vi "DialogManageInterfaces.vi"(8 "error in (no error)":errorcluster, 10 "ClassItemRefIn":refnum<vi>, 11 "ClassWriterNativeIn":refnum<class "ClassWriterNative.lvclass">) -> (0 "error out":errorcluster, 1 "HanldeInterfacesData":T1, 2 "Cancelled":bool, 3 "ClassWriterNativeOut":refnum<class "ClassWriterNative.lvclass">)   [LabVIEW 2020, in "ClassWriterNative.lvclass"]
uses:
  <resource>/Framework/Providers/Open_GDS/ClassProviders/Provider_LvNativeClass/ClassWriterNative_class/ClassWriterNative.lvclass
  <resource>/Framework/Providers/Open_GDS/ClassProviders/Provider_BaseClassInterface/ClassWriter_class/HandleInterfacesData.ctl
  <resource>/Framework/Providers/Open_GDS/ClassProviders/Common/InterfaceLibrary/InterfaceInfo.ctl
  <resource>/Framework/Providers/Open_GDS/ClassProviders/Common/LvClass_class/GDSLvClass_ClassMethodInfo.ctl
  <resource>/Framework/Providers/Open_GDS/ClassProviders/Provider_BaseClassInterface/ClassWriter_class/InterfacesToImplement.ctl
  <resource>/Framework/Providers/Open_GDS/ClassProviders/Common/LvClass_class/GDSLvClass_ClassInfo.ctl
  <vilib>/picture/picture.llb/imagedata.ctl
  <vilib>/Utility/miscctls.llb/LVRowAndColumnTypeDef.ctl
  <vilib>/Utility/miscctls.llb/LVRowAndColumnUnsignedTypeDef.ctl
  faae8295-b5d0-4054-ba26-443edd8c351b.vi
  a5869a5e-804e-44c9-8055-a166d2e26855.vi
  516f7541-512c-4146-8a63-54cd49fe1b68.vi
  c799aba2-3e95-4f13-9023-21e7452f1ffd.vi
  <resource>/Framework/Providers/Open_GDS/ClassProviders/Provider_LvNativeClass/ClassWriterNative_class/ClassWriterNative.lvclass/ClassWriterNative.ctl
  <resource>/Framework/Providers/Open_GDS/ClassProviders/Common/InterfaceLibrary/InterfaceLibrary.lvlib
  <resource>/Framework/Providers/Open_GDS/ClassProviders/Provider_BaseClassInterface/ClassWriter_class/ClassWriter.lvclass
  <resource>/Framework/Providers/_ClassSupport/Class Provider Support.lvlib
panel:
  in  "Tree":string(tree) caption="No methods selected"
  in  "_ShowContextHelp":bool
  in  "Help":bool
  in  "Cancel":bool
  in  "Save":bool
  out "ProductPicture":picture
  out "InterfaceList":i32[](listbox)
  in  "InterfaceFilter":string caption="Filter"
  out "Class":string
  # "Select Parent Interfaces (tick or untick check box)"
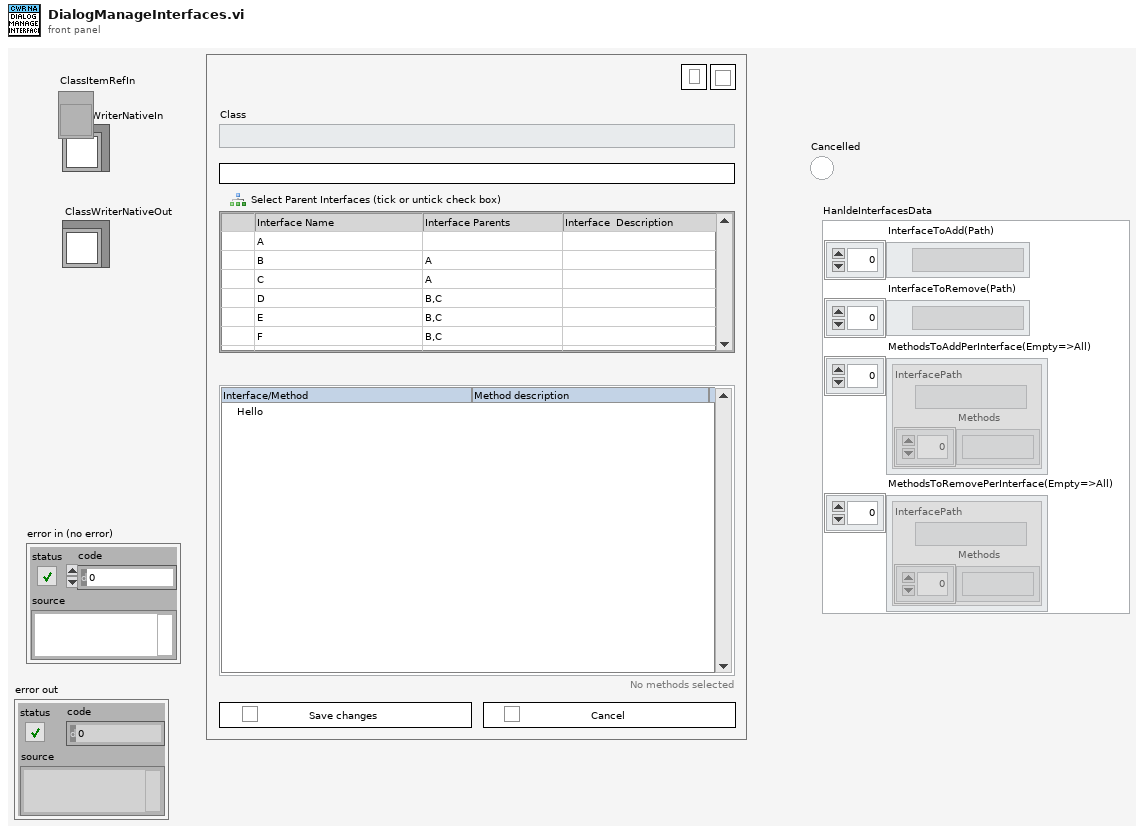
[diagram p1: front panel]
types:
  T1 = typedef "ClassWriter.lvclass/HandleInterfacesData.ctl" = cluster{"InterfaceToAdd(Path)":path[], "InterfaceToRemove(Path)":path[], "MethodsToAddPerInterface(Empty=>All)":cluster{"InterfacePath":path, "Methods":string[]}[], "MethodsToRemovePerInterface(Empty=>All)":cluster{"InterfacePath":path, "Methods":string[]}[]}
  T2 = cluster{"Font Name":string, "Size":u16, "Bold":bool, "Italic":bool, "Underline":bool, "Strikeout":bool, "Color":u32}
  T3 = typedef "InterfaceLibrary.lvlib/InterfaceInfo.ctl" = cluster{"Name(Short if no Conflicts)":string, "FullQualifierName":string, "Description":string, "Path":path, "ParentInterfaceNames(Short if no Conflitcs)":string[], "ParentInterfaceFullQualifierNames":string[], "IconPath":path, "Methods":T4[], "DynamicDispatchMethod":bool[]}
  T4 = typedef "GDSLvClass_ClassMethodInfo.ctl" = cluster{"Name":string, "Descriptions":string, "RelativePath":path, "SourceScope":enum32{"invalid scope", "public", "private", "protected", "community"}, "MustOverride":bool, "VirtualFolderLocation":string[], "DynamicDispatch":bool}
  T5 = typedef "ClassWriter.lvclass/InterfacesToImplement.ctl" = cluster{"InterfacePath":path[], "CreateMethods":bool, "MethodsPerInterface(Empty=>All)":cluster{"Methods":string[]}[]}
  T6 = typedef "GDSLvClass_ClassInfo.ctl" = cluster{"Path":path, "Name":string, "QualifiedName":string}
  T7 = cluster{"Cancel":bool, "InterfaceInfo":T3[], "IsInterface?":bool, "ParentInterfaces(path)":path[], "Interfaces(MethodsImplemented)":cluster{"Methods":string[]}[], "InterfaceIcons":path[], "VisiableInterfaceIndexes":i32[], "InterfaceSelection":enum16{"Empty", "Not", "Grey", "Blue"}[], "DisabledInterfaceIndexes":i32[], "InterfaceToAdd":T5, "InterfaceToRemove":T5, "MethodsSelectedPerInt":cluster{"Array":bool[]}[], "MethodsPerInterfaces":cluster{"Array":string[]}[], "Interfaces":string[], "StartInterfaceSelection":bool[], "Path":path, "DisabledInterafaces":i32[], "MethodsDisabledPerInt":cluster{"Array":bool[]}[], "SelectedInterfaceIndex":i32[], "ClassInheritanceHierarchy":T6[], "InterfacesParentClasesUses(path)":path[], "LvClasses":refnum<vi>[], "LvInterfaces":refnum<vi>[], "HandleInterfacesData":T1}
  T8 = typedef "imagedata.ctl" = cluster{"image type":i32, "image depth":i32, "image":u8[], "mask":u8[], "colors":u32[], "Rectangle":cluster{"left":i16, "top":i16, "right":i16, "bottom":i16}}
  T9 = typedef "LVRowAndColumnTypeDef.ctl" = cluster{"Row":i32, "Column":i32}
  T10 = typedef "LVRowAndColumnUnsignedTypeDef.ctl" = cluster{"Row":u32, "Column":u32}
  T11 = cluster{"FullQualifierInterfaceName":string, "MethodNames":string[]}[]
  T12 = cluster{"InterfacePath":path, "Methods":string[]}
  T13 = cluster{"ParentInterfaceFullQualifierNames":string[]}
  T14 = cluster{"FullQualifierName":string, "Methods":string[]}
  T15 = typedef "LVPoint32TypeDef.ctl" = cluster{"Horizontal":i32, "Vertical":i32}
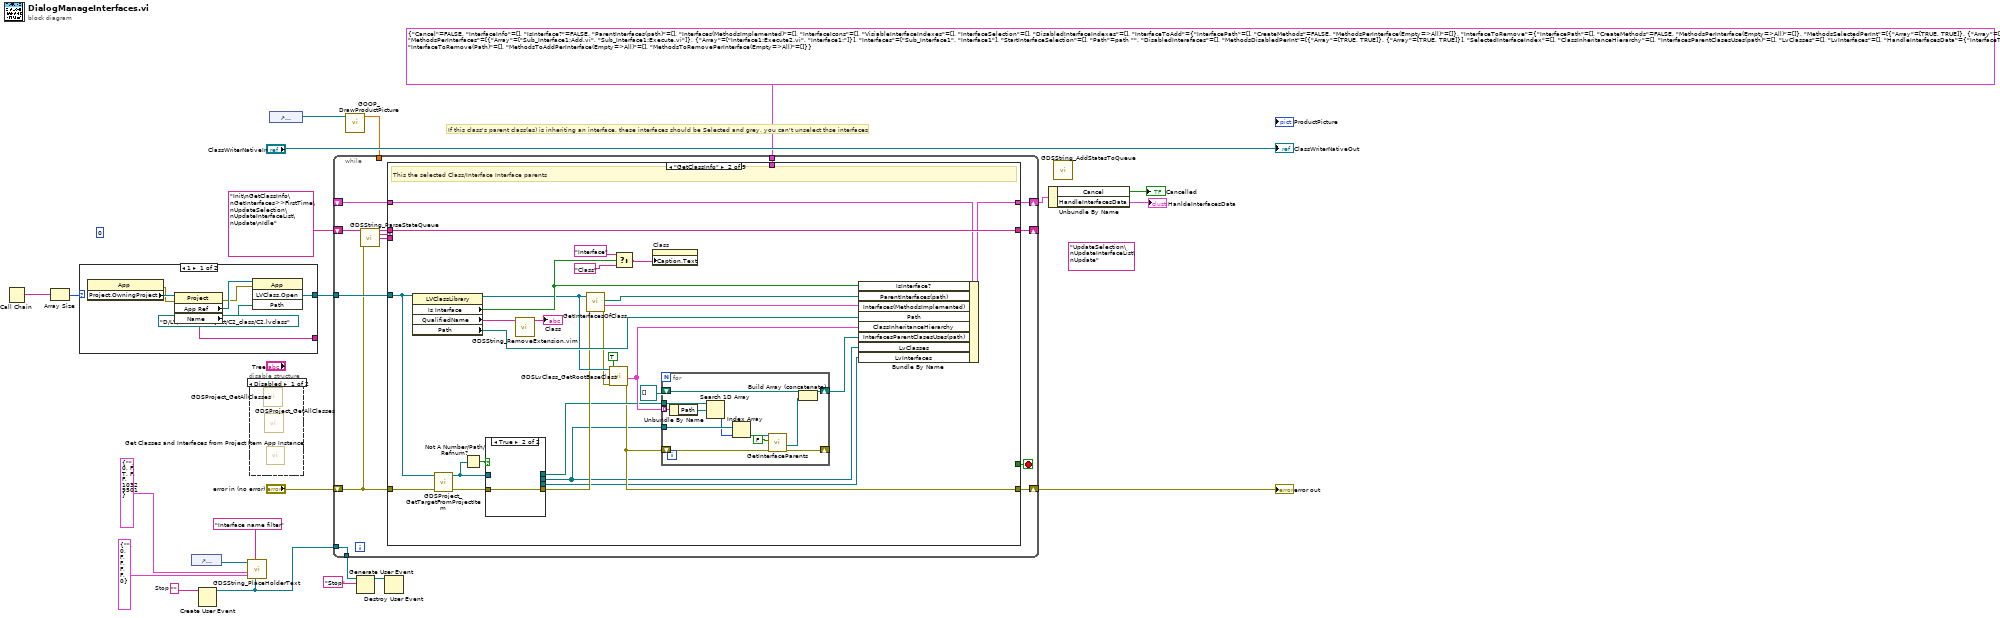
[diagram p0: block diagram]
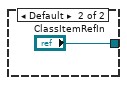
[diagram p3: hidden frame]
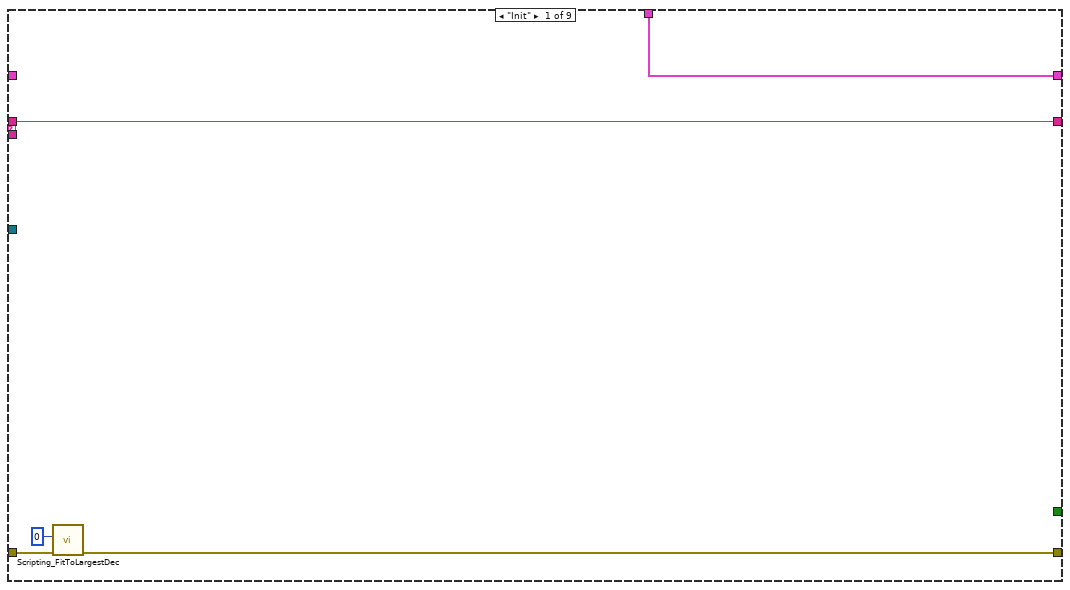
[diagram p4: hidden frame]
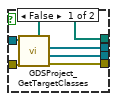
[diagram p5: hidden frame]
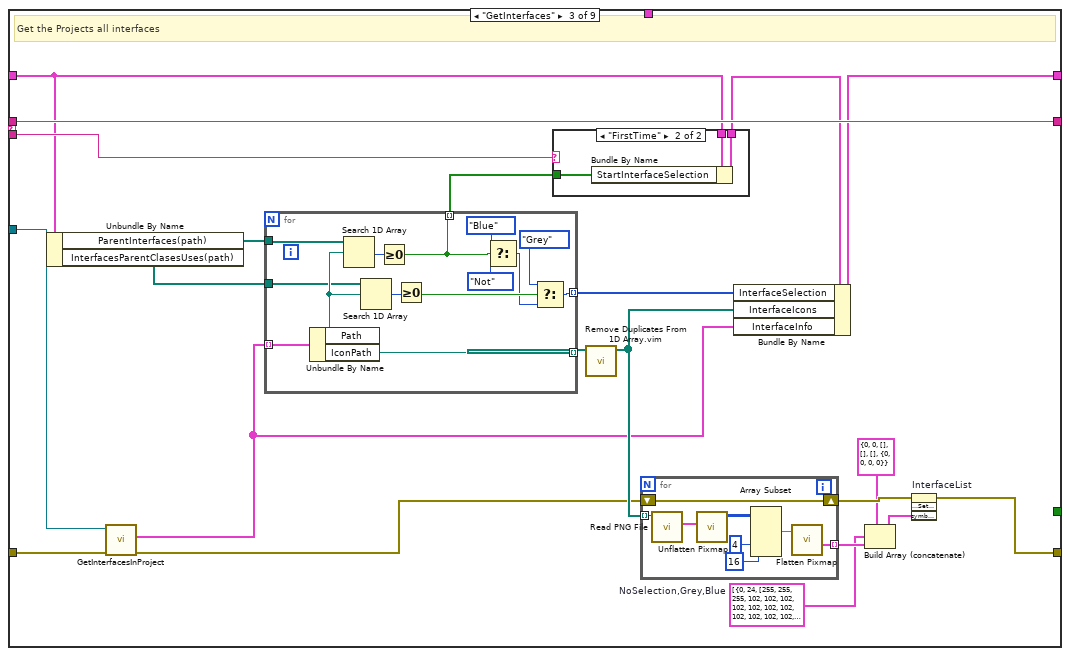
[diagram p6: hidden frame]
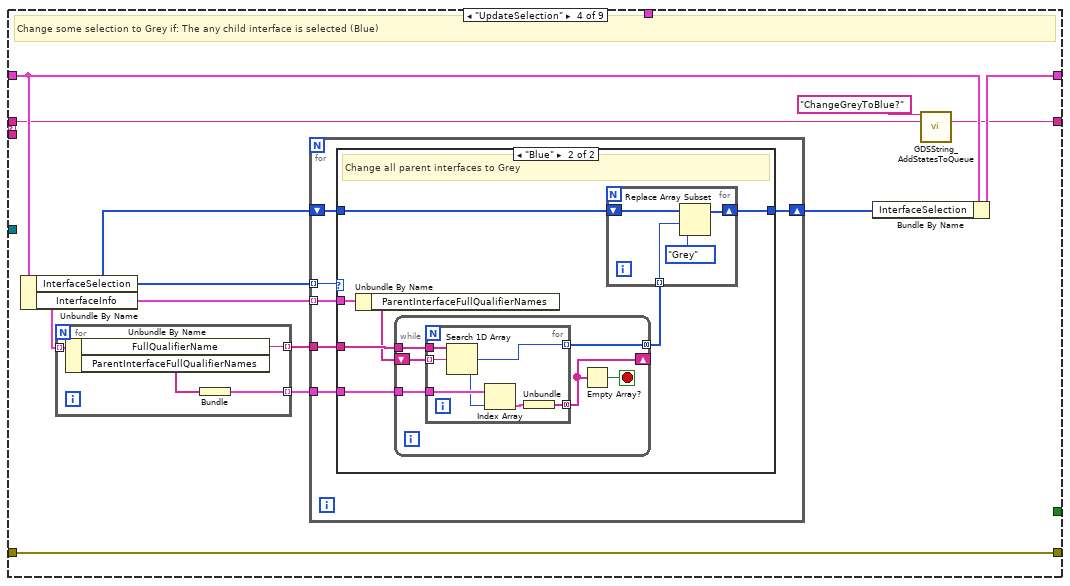
[diagram p8: hidden frame]
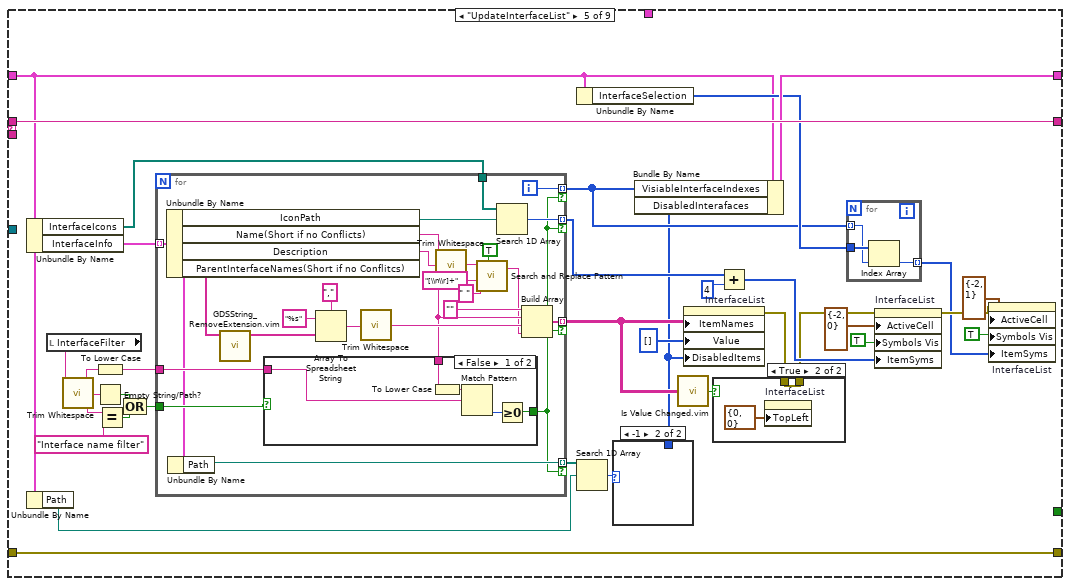
[diagram p10: hidden frame]
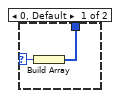
[diagram p11: hidden frame]
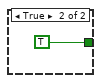
[diagram p13: hidden frame]
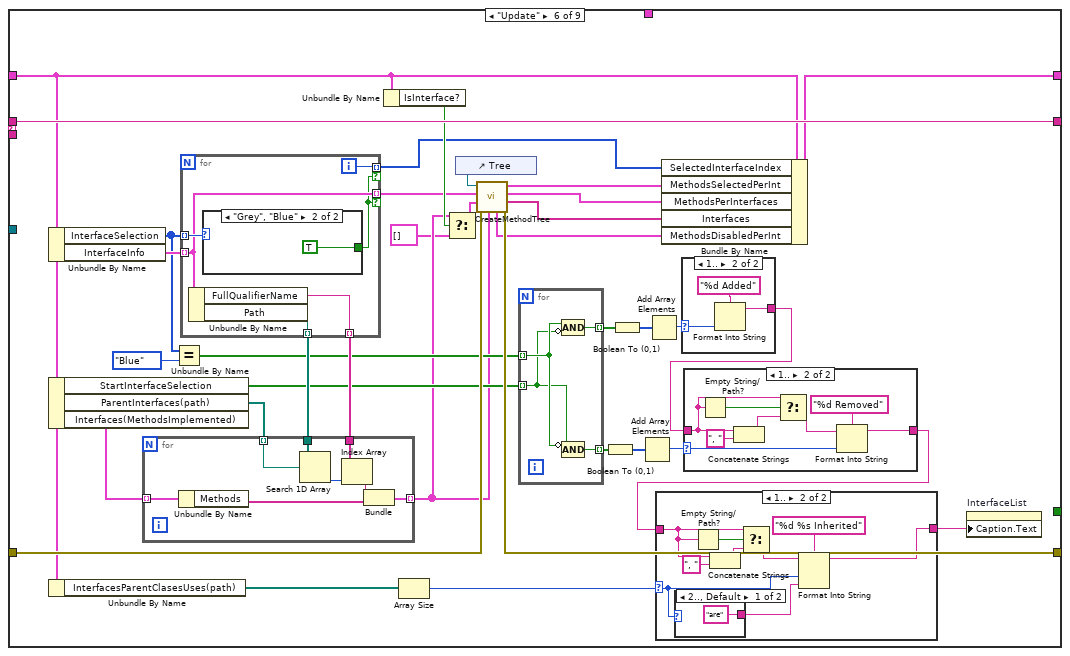
[diagram p14: hidden frame]
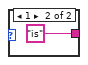
[diagram p16: hidden frame]
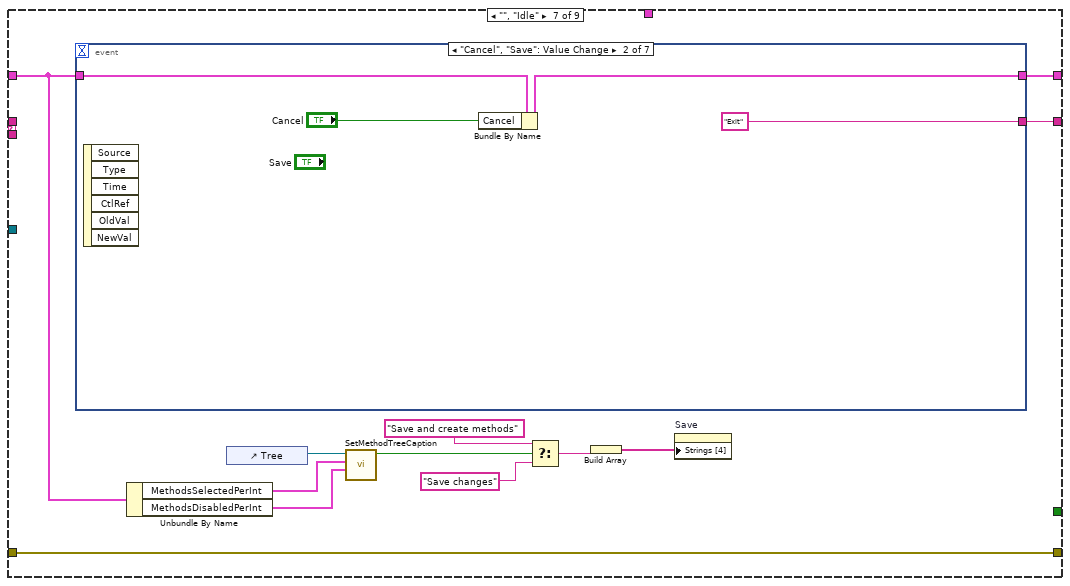
[diagram p20: hidden frame]
diagram:
  (unwired) 0
  w6 = ""  # Stop
  (unwired) "UpdateSelection\nUpdateInterfaceList\nUpdate"
  # "If this class's parent class(es) is inheriting an interface, these interfaces should be Selected and grey, you can't unselect thse interfaces"
  n1 = Call Chain() -> (call chain=w4:string[])
  n2 = Array Size(array=w4) -> (size(s)=w2:i32)
  n3 = case shown="1" w2 {
    tunnel: [w29 "ClassItemRefIn"] -> w9
    tunnel: [w23 _] -> _
    frame 1 {
      n4 = property class="App"() -> (error out=w25:errorcluster, "Project.OwningProject"=w26:refnum<vi>)  [unwired: 2 in, 1 out]
      n5 = property class="Project"(reference=w26, error in=w25) -> (error out=w24:errorcluster, "App Ref"=w27:refnum<vi>, "Name"=w23:string)  [unwired: 1 out]
      n6 = invoke class="App" method="LVClass.Open"(reference=w27, error in=w24, "Path"=path "D:/LV/RenameProject/C2_class/C2.lvclass") -> ("LVClass.Open"=w29:refnum<vi>)  [unwired: 1 in, 3 out]
    }
    frame Default {
    }
  }
  n7 = control-ref of="InterfaceFilter"() -> (w10:refnum<vi>)
  n8 = Create User Event(user event datatype=w6) -> (user event=w12:refnum<user-event>)  [unwired: 1 in, 1 out]
  n9 = call <resource>:"GDSString_PlaceHolderText.vi"("BooleanUserEventToStopPlaceHolderVI"=w12, "PlaceholderText"="Interface name filter" ("InterfaceFilter"), "PlaceholderTextFont(Grey,Italic)"=T2 {"Font Name"="", "Size"=0, "Bold"=FALSE, "Italic"=TRUE, "Underline"=FALSE, "Strikeout"=FALSE, "Color"=10329501}, "NormalTextFont(Black)"=T2 {"Font Name"="", "Size"=0, "Bold"=FALSE, "Italic"=FALSE, "Underline"=FALSE, "Strikeout"=FALSE, "Color"=0}, "PlaceholderStringRef"=w10) -> ()  [unwired: 6 in, 1 out]
  n10 = disable-structure shown="Disabled" {
    frame Disabled {
      n11 = call <resource>:"GDSProject_GetAllClasses.vi"() -> ()  [unwired: 17 in, 3 out]
      n12 = call <resource>:"GDSProject_GetAllClasses.vi"() -> ()  [unwired: 17 in, 3 out]
      n13 = call <resource>:"Get Classes and Interfaces from Project Item App Instance.vi"() -> ()  [unwired: 5 in, 7 out]
    }
    frame Enabled {
    }
  }
  n14 = control-ref of="ProductPicture"() -> (w18:refnum<vi>)
  n15 = call <resource>:"GOOP_DrawProductPicture.vi"("ProductPictureControl"=w18) -> ("Zoom Factor"=w17:sgl)  [unwired: 10 in]
  n16 = while {
    shift-right: [w42] -> w21
    shift-left: "error in (no error)" -> [w33]
    shift-right: [w39] -> _
    shift-left: "Init\nGetClassInfo\nGetInterfaces>>FirstTime\nUpdateSelection\nUpdateInterfaceList\nUpdate\nIdle" -> [w41]
    tunnel: T7 {"Cancel"=FALSE, "InterfaceInfo"=[], "IsInterface?"=FALSE, "ParentInterfaces(path)"=[], "Interfaces(MethodsImplemented)"=[], "InterfaceIcons"=[], "VisiableInterfaceIndexes"=[], "InterfaceSelection"=[], "DisabledInterfaceIndexes"=[], "InterfaceToAdd"={"InterfacePath"=[], "CreateMethods"=FALSE, "MethodsPerInterface(Empty=>All)"=[]}, "InterfaceToRemove"={"InterfacePath"=[], "CreateMethods"=FALSE, "MethodsPerInterface(Empty=>All)"=[]}, "MethodsSelectedPerInt"=[{"Array"=[TRUE, TRUE]}, {"Array"=[TRUE, TRUE]}], "MethodsPerInterfaces"=[{"Array"=["Sub_Interface1:Add.vi", "Sub_Interface1:Execute.vi"]}, {"Array"=["Interface1:Execute2.vi", "Interface1:"]}], "Interfaces"=["Sub_Interface1", "Interface1"], "StartInterfaceSelection"=[], "Path"=path "", "DisabledInterafaces"=[], "MethodsDisabledPerInt"=[{"Array"=[TRUE, TRUE]}, {"Array"=[TRUE, TRUE]}], "SelectedInterfaceIndex"=[], "ClassInheritanceHierarchy"=[], "InterfacesParentClasesUses(path)"=[], "LvClasses"=[], "LvInterfaces"=[], "HandleInterfacesData"={"InterfaceToAdd(Path)"=[], "InterfaceToRemove(Path)"=[], "MethodsToAddPerInterface(Empty=>All)"=[], "MethodsToRemovePerInterface(Empty=>All)"=[]}} -> [w36]
    shift-right: [w37] -> w8
    shift-left: _ -> [w35]
    tunnel: w9 -> [w34]
    tunnel: w17 -> [_]
    tunnel: w12 -> [w32]
    tunnel: [w32] -> w11
    stop <- w38 stop-if-true
    n17 = call <resource>:"GDSString_ParseStateQueue.vi"("State Queue"=w41, "Error In (no error)"=w33) -> ("Remaining States"=w40:string, "Current State"=w43:string, "Arguments"=w31:string)  [unwired: 9 in, 2 out]
    n18 = case shown="\"GetClassInfo\"" w43 {
      tunnel: [w45 w58 w107 w153 w220 w291 w347 w414 w480] -> w42
      tunnel: w33 -> [w46 w61 w115 w153 w220 w290 w347 w414 w480]
      tunnel: [w44 w76 w116 w144 w219 w294 w349 w409 w481] -> w39
      tunnel: w40 -> [w44 w76 w116 w145 w219 w294 _ w410 w481]
      tunnel: [_ _ _ _ _ _ _ _ TRUE] -> w38
      tunnel: [w48 w74 w113 w151 w203 w289 w348 w412 w478] -> w37
      tunnel: w36 -> [w48 _ _ _ _ _ _ _ _]
      tunnel: w35 -> [_ w75 w100 w152 w193 w263 w345 w413 w471]
      tunnel: w34 -> [_ w52 w114 _ _ _ _ _ _]
      tunnel: w31 -> [_ _ w101 _ _ _ _ _ _]
      frame "Init" {
        n19 = call <resource>:"Scripting_FitToLargestDec.vi"("error in (no error)"=w46, "border spacing (2 px)"=0) -> ("error out"=w45:errorcluster)  [unwired: 4 in, 1 out]
      }
      frame "GetClassInfo" {
        # "This the selected Class/Interface Interface parents"
        n20 = property class="LVClassLibrary"(reference=w52) -> (reference out=w64:refnum<vi>, "Is Interface"=w71:bool, "QualifiedName"=w67:string, "Path"=w65:path)  [unwired: 1 in, 1 out]
        n21 = call <resource>:"GDSProject_GetTargetFromProjectItem.vi"("error in (no error)"=w61, "ProjectItem in"=w52) -> ("error out"=w51:errorcluster, "TargetItem out"=w50:refnum<vi>)  [unwired: 8 in]
        n22 = Not A Number/Path/Refnum?(number/path/refnum=w50) -> (NaN/Path/Refnum?=w49:bool)
        n23 = case shown="True" w49 {
          tunnel: [w82 w83] -> w62
          tunnel: [w81 _] -> w59
          tunnel: [w80 _] -> w55
          tunnel: [w79 _] -> w54
          tunnel: w51 -> [w78 w83]
          tunnel: w50 -> [w77 _]
          frame False {
            n24 = call <resource>:"GDSProject_GetTargetClasses.vi"("error in (no error)"=w78, "TargetItem in"=w77) -> ("error out"=w82:errorcluster, "LvInterfaces"=w79:refnum<vi>[], "LvClasses"=w80:refnum<vi>[], "LvClasses(Path)"=w81:path[])  [unwired: 4 in, 2 out]
          }
          frame True {
          }
        }
        n25 = call "GDSString_RemoveExtension.vim"("NameWithExtension"=w67) -> ("NameWithoutExtension"=→"Class":string)  [unwired: 9 in, 1 out]
        n26 = call <resource>:"GetInterfacesOfClass.vi"("error in"=w62, "LvClassRefIn"=w64) -> ("error out"=w63:errorcluster, "Interfaces(MethodsImplemented)"=w72:cluster{"Methods":string[]}[], "Interfaces(path)"=w73:path[])  [unwired: 6 in, 1 out]
        n27 = call <resource>:"GDSLvClass_GetRootBaseClass.vi"("ViRef/Path,LvClassRef/Path"=w64, "error in (no error)"=w63, "Don'tOpenReference"=TRUE) -> ("InheritanceHierarchy"=w60:T6[], "error out"=w58:errorcluster)  [unwired: 10 in, 5 out]
        n28 = Select(t="Interface", s=w71, f="Class") -> (s? t:f=w70:string)
        n29 = property on="Class" class="Str"("Caption.Text"=w70) -> ()  [unwired: 2 in, 2 out]
        n30 = for {
          tunnel: w60 -> [w95] mode=indexing
          tunnel: w59 -> [w93]
          tunnel: w55 -> [w92]
          shift-right: [w87] -> _
          shift-left: w58 -> [w88]
          shift-right: [w89] -> w56
          shift-left: path[] [] -> [w90]
          n31 = Unbundle By Name(w95) -> ("Path"=w94:path)
          n32 = Search 1D Array(1D array=w93, element=w94) -> (index of element=w91:i32)  [unwired: 1 in]
          n33 = Index Array(array=w92, index=w91) -> (element=w86:refnum<vi>)
          n34 = call <resource>:"GetInterfaceParents.vi"("error in (no error)"=w88, "KeepRefsOpen"=FALSE, "LVClassLibrary in"=w86) -> ("error out"=w87:errorcluster, "InterfaceParents(Path)"=w84:path[])  [unwired: 5 in, 2 out]
          n35 = Build Array (concatenate)(w90, w84) -> (w89:path[])
        }
        n36 = Bundle By Name(cluster=w75, "IsInterface?"=w71, "ParentInterfaces(path)"=w73, "Interfaces(MethodsImplemented)"=w72, "Path"=w65, "ClassInheritanceHierarchy"=w60, "InterfacesParentClasesUses(path)"=w56, "LvClasses"=w55, "LvInterfaces"=w54) -> (w74:T7)
      }
      frame "GetInterfaces" {
        w102 = T8[] [{"image type"=0, "image depth"=24, "image"=[255, 255, 255, 102, 102, 102, 102, 102, 102, 102, 102, 102, 102, 102, 102, 102, 102, 102, 102, 102, 102, 102, 102, 102, 102, 102, 102, 102, 102, 102, 102, 102, 102, 102, 102, 102, 255, 255, 255, 102, 102, 102, 102, 102, 102, 102, 102, 102, 102, 102, 102, 102, 102, 102, 102, 102, 102, 102, 102, 102, 102, 102, 102, 102, 102, 102, 102, 102, 102, 102, 102, 102, 102, 102, 102, 102, 102, 102, 102, 102, 102, 102, 102, 102, 255, 255, 255, 255, 255, 255, 255, 255, 255, 255, 255, 255, 255, 255, 255, 255, 255, 255, 255, 255, 255, 255, 255, 255, 255, 255, 255, 102, 102, 102, 102, 102, 102, 102, 102, 102, 102, 102, 102, 255, 255, 255, 255, 255, 255, 255, 255, 255, 255, 255, 255, 255, 255, 255, 255, 255, 255, 255, 255, 255, 255, 255, 255, 255, 255, 255, 102, 102, 102, 102, 102, 102, 102, 102, 102, 102, 102, 102, 255, 255, 255, 255, 255, 255, 255, 255, 255, 255, 255, 255, 255, 255, 255, 255, 255, 255, 255, 255, 255, 255, 255, 255, 255, 255, 255, 102, 102, 102, 102, 102, 102, 102, 102, 102, 102, 102, 102, 255, 255, 255, 255, 255, 255, 255, 255, 255, 255, 255, 255, 255, 255, 255, 255, 255, 255, 255, 255, 255, 255, 255, 255, 255, 255, 255, 102, 102, 102, 102, 102, 102, 102, 102, 102, 102, 102, 102, 255, 255, 255, 255, 255, 255, 255, 255, 255, 255, 255, 255, 255, 255, 255, 255, 255, 255, 255, 255, 255, 255, 255, 255, 255, 255, 255, 102, 102, 102, 102, 102, 102, 102, 102, 102, 102, 102, 102, 255, 255, 255, 255, 255, 255, 255, 255, 255, 255, 255, 255, 255, 255, 255, 255, 255, 255, 255, 255, 255, 255, 255, 255, 255, 255, 255, 102, 102, 102, 102, 102, 102, 102, 102, 102, 102, 102, 102, 255, 255, 255, 255, 255, 255, 255, 255, 255, 255, 255, 255, 255, 255, 255, 255, 255, 255, 255, 255, 255, 255, 255, 255, 255, 255, 255, 102, 102, 102, 102, 102, 102, 102, 102, 102, 102, 102, 102, 255, 255, 255, 255, 255, 255, 255, 255, 255, 255, 255, 255, 255, 255, 255, 255, 255, 255, 255, 255, 255, 255, 255, 255, 255, 255, 255, 102, 102, 102, 102, 102, 102, 102, 102, 102, 102, 102, 102, 255, 255, 255, 255, 255, 255, 255, 255, 255, 255, 255, 255, 255, 255, 255, 255, 255, 255, 255, 255, 255, 255, 255, 255, 255, 255, 255, 102, 102, 102, 102, 102, 102, 102, 102, 102, 102, 102, 102, 102, 102, 102, 102, 102, 102, 102, 102, 102, 102, 102, 102, 102, 102, 102, 102, 102, 102, 102, 102, 102, 102, 102, 102, 102, 102, 102, 102, 102, 102, 102, 102, 102, 255, 255, 255, 102, 102, 102, 102, 102, 102, 102, 102, 102, 102, 102, 102, 102, 102, 102, 102, 102, 102, 102, 102, 102, 102, 102, 102, 102, 102, 102, 102, 102, 102, 102, 102, 102, 255, 255, 255], "mask"=[255, 248, 255, 248, 255, 248, 255, 248, 255, 248, 255, 248, 255, 248, 255, 248, 255, 248, 255, 248, 255, 248, 255, 248, 255, 248], "colors"=[], "Rectangle"={"left"=0, "top"=0, "right"=13, "bottom"=13}}, {"image type"=0, "image depth"=24, "image"=[255, 255, 255, 143, 143, 143, 143, 143, 143, 143, 143, 143, 143, 143, 143, 143, 143, 143, 143, 143, 143, 143, 143, 143, 143, 143, 143, 143, 143, 143, 143, 143, 143, 143, 143, 143, 255, 255, 255, 143, 143, 143, 143, 143, 143, 143, 143, 143, 143, 143, 143, 143, 143, 143, 143, 143, 143, 143, 143, 143, 143, 143, 143, 143, 143, 143, 143, 143, 143, 143, 143, 143, 170, 170, 170, 143, 143, 143, 143, 143, 143, 143, 143, 143, 143, 143, 143, 143, 143, 143, 143, 143, 143, 143, 143, 143, 143, 143, 143, 143, 143, 143, 143, 143, 143, 143, 143, 143, 170, 170, 170, 211, 211, 211, 143, 143, 143, 143, 143, 143, 143, 143, 143, 143, 143, 143, 143, 143, 143, 143, 143, 143, 143, 143, 143, 143, 143, 143, 143, 143, 143, 143, 143, 143, 170, 170, 170, 232, 232, 232, 255, 255, 255, 143, 143, 143, 143, 143, 143, 143, 143, 143, 143, 143, 143, 143, 143, 143, 143, 143, 143, 143, 143, 143, 143, 143, 143, 143, 143, 143, 170, 170, 170, 232, 232, 232, 255, 255, 255, 211, 211, 211, 143, 143, 143, 143, 143, 143, 143, 143, 143, 158, 158, 158, 143, 143, 143, 143, 143, 143, 143, 143, 143, 143, 143, 143, 170, 170, 170, 232, 232, 232, 255, 255, 255, 211, 211, 211, 143, 143, 143, 143, 143, 143, 143, 143, 143, 211, 211, 211, 218, 218, 218, 158, 158, 158, 143, 143, 143, 143, 143, 143, 170, 170, 170, 232, 232, 232, 255, 255, 255, 211, 211, 211, 154, 154, 154, 143, 143, 143, 143, 143, 143, 143, 143, 143, 226, 226, 226, 255, 255, 255, 218, 218, 218, 158, 158, 158, 170, 170, 170, 232, 232, 232, 255, 255, 255, 211, 211, 211, 154, 154, 154, 143, 143, 143, 143, 143, 143, 143, 143, 143, 143, 143, 143, 165, 165, 165, 226, 226, 226, 255, 255, 255, 218, 218, 218, 232, 232, 232, 255, 255, 255, 211, 211, 211, 154, 154, 154, 143, 143, 143, 143, 143, 143, 143, 143, 143, 143, 143, 143, 143, 143, 143, 143, 143, 143, 165, 165, 165, 226, 226, 226, 255, 255, 255, 255, 255, 255, 211, 211, 211, 154, 154, 154, 143, 143, 143, 143, 143, 143, 143, 143, 143, 143, 143, 143, 143, 143, 143, 143, 143, 143, 143, 143, 143, 143, 143, 143, 165, 165, 165, 226, 226, 226, 211, 211, 211, 154, 154, 154, 143, 143, 143, 143, 143, 143, 143, 143, 143, 143, 143, 143, 143, 143, 143, 143, 143, 143, 143, 143, 143, 143, 143, 143, 143, 143, 143, 143, 143, 143, 165, 165, 165, 154, 154, 154, 143, 143, 143, 143, 143, 143, 143, 143, 143, 143, 143, 143, 143, 143, 143, 143, 143, 143, 143, 143, 143, 255, 255, 255, 143, 143, 143, 143, 143, 143, 143, 143, 143, 143, 143, 143, 143, 143, 143, 143, 143, 143, 143, 143, 143, 143, 143, 143, 143, 143, 143, 143, 143, 143, 143, 143, 143, 255, 255, 255], "mask"=[255, 248, 255, 248, 255, 248, 255, 248, 255, 248, 255, 248, 255, 248, 255, 248, 255, 248, 255, 248, 255, 248, 255, 248, 255, 248], "colors"=[], "Rectangle"={"left"=0, "top"=0, "right"=13, "bottom"=13}}, {"image type"=0, "image depth"=24, "image"=[255, 255, 255, 33, 150, 243, 33, 150, 243, 33, 150, 243, 33, 150, 243, 33, 150, 243, 33, 150, 243, 33, 150, 243, 33, 150, 243, 33, 150, 243, 33, 150, 243, 33, 150, 243, 255, 255, 255, 33, 150, 243, 33, 150, 243, 33, 150, 243, 33, 150, 243, 33, 150, 243, 33, 150, 243, 33, 150, 243, 33, 150, 243, 33, 150, 243, 33, 150, 243, 33, 150, 243, 93, 178, 246, 33, 150, 243, 33, 150, 243, 33, 150, 243, 33, 150, 243, 33, 150, 243, 33, 150, 243, 33, 150, 243, 33, 150, 243, 33, 150, 243, 33, 150, 243, 33, 150, 243, 93, 178, 246, 174, 217, 251, 33, 150, 243, 33, 150, 243, 33, 150, 243, 33, 150, 243, 33, 150, 243, 33, 150, 243, 33, 150, 243, 33, 150, 243, 33, 150, 243, 33, 150, 243, 93, 178, 246, 214, 236, 253, 255, 255, 255, 33, 150, 243, 33, 150, 243, 33, 150, 243, 33, 150, 243, 33, 150, 243, 33, 150, 243, 33, 150, 243, 33, 150, 243, 33, 150, 243, 93, 178, 246, 214, 236, 253, 255, 255, 255, 174, 217, 251, 33, 150, 243, 33, 150, 243, 33, 150, 243, 67, 166, 245, 33, 150, 243, 33, 150, 243, 33, 150, 243, 33, 150, 243, 93, 178, 246, 214, 236, 253, 255, 255, 255, 174, 217, 251, 33, 150, 243, 33, 150, 243, 33, 150, 243, 174, 217, 251, 187, 223, 251, 67, 166, 245, 33, 150, 243, 33, 150, 243, 93, 178, 246, 214, 236, 253, 255, 255, 255, 174, 217, 251, 58, 162, 244, 33, 150, 243, 33, 150, 243, 33, 150, 243, 203, 230, 252, 255, 255, 255, 187, 223, 251, 67, 166, 245, 93, 178, 246, 214, 236, 253, 255, 255, 255, 174, 217, 251, 58, 162, 244, 33, 150, 243, 33, 150, 243, 33, 150, 243, 33, 150, 243, 82, 173, 246, 203, 230, 252, 255, 255, 255, 187, 223, 251, 214, 236, 253, 255, 255, 255, 174, 217, 251, 58, 162, 244, 33, 150, 243, 33, 150, 243, 33, 150, 243, 33, 150, 243, 33, 150, 243, 33, 150, 243, 82, 173, 246, 203, 230, 252, 255, 255, 255, 255, 255, 255, 174, 217, 251, 58, 162, 244, 33, 150, 243, 33, 150, 243, 33, 150, 243, 33, 150, 243, 33, 150, 243, 33, 150, 243, 33, 150, 243, 33, 150, 243, 82, 173, 246, 203, 230, 252, 174, 217, 251, 58, 162, 244, 33, 150, 243, 33, 150, 243, 33, 150, 243, 33, 150, 243, 33, 150, 243, 33, 150, 243, 33, 150, 243, 33, 150, 243, 33, 150, 243, 33, 150, 243, 82, 173, 246, 58, 162, 244, 33, 150, 243, 33, 150, 243, 33, 150, 243, 33, 150, 243, 33, 150, 243, 33, 150, 243, 33, 150, 243, 255, 255, 255, 33, 150, 243, 33, 150, 243, 33, 150, 243, 33, 150, 243, 33, 150, 243, 33, 150, 243, 33, 150, 243, 33, 150, 243, 33, 150, 243, 33, 150, 243, 33, 150, 243, 255, 255, 255], "mask"=[255, 248, 255, 248, 255, 248, 255, 248, 255, 248, 255, 248, 255, 248, 255, 248, 255, 248, 255, 248, 255, 248, 255, 248, 255, 248], "colors"=[], "Rectangle"={"left"=0, "top"=0, "right"=13, "bottom"=13}}]  # NoSelection,Grey,Blue
        # "Get the Projects all interfaces"
        n37 = Unbundle By Name(w100) -> ("ParentInterfaces(path)"=w105:path[], "InterfacesParentClasesUses(path)"=w97:path[])
        n38 = call <resource>:"GetInterfacesInProject.vi"("error in"=w115, "Project/ProjectItem"=w114) -> ("error out"=w108:errorcluster, "InterfaceInfo"=w96:T3[])  [unwired: 8 in]
        n39 = for {
          tunnel: w96 -> [w142] mode=indexing
          tunnel: [w141] -> w110 mode=indexing
          tunnel: w105 -> [w140]
          tunnel: [w131] -> w104 mode=indexing
          tunnel: [w129] -> w98 mode=indexing
          tunnel: w97 -> [w135]
          n40 = Unbundle By Name(w142) -> ("Path"=w136:path, "IconPath"=w141:path)
          n41 = Search 1D Array(1D array=w140, element=w136) -> (index of element=w139:i32)  [unwired: 1 in]
          n42 = Search 1D Array(1D array=w135, element=w136) -> (index of element=w134:i32)  [unwired: 1 in]
          n43 = Greater Or Equal To 0?(x=w139) -> (x >= 0?=w129:bool)
          n44 = Greater Or Equal To 0?(x=w134) -> (x >= 0?=w133:bool)
          n45 = Select(t=enum16{"Empty", "Not", "Grey", "Blue"}."Blue", s=w129, f=enum16{"Empty", "Not", "Grey", "Blue"}."Not") -> (s? t:f=w132:enum16{"Empty", "Not", "Grey", "Blue"})
          n46 = Select(t=enum16{"Empty", "Not", "Grey", "Blue"}."Grey", s=w133, f=w132) -> (s? t:f=w131:enum16{"Empty", "Not", "Grey", "Blue"})
        }
        n47 = case shown="\"FirstTime\"" w101 {
          tunnel: w100 -> [w117 w120]
          tunnel: [w117 w119] -> w99
          tunnel: w98 -> [_ w118]
          frame Default {
          }
          frame "FirstTime" {
            n48 = Bundle By Name(cluster=w120, "StartInterfaceSelection"=w118) -> (w119:T7)
          }
        }
        n49 = call "Remove Duplicates From 1D Array.vim"("array"=w110) -> ("array with duplicates removed"=w109:path[])  [unwired: 10 in]
        n50 = for {
          tunnel: w109 -> [w128] mode=indexing
          shift-right: [w122] -> w111
          shift-left: w108 -> [w122]
          tunnel: [w121] -> w112 mode=indexing
          n51 = call <vilib>:"Read PNG File.vi"("path to PNG file"=w128) -> ("image data"=w127:T8)  [unwired: 8 in, 2 out]
          n52 = call <vilib>:"Unflatten Pixmap.vi"("image data"=w127) -> ("24-bit pixmap"=w126:u32[][])  [unwired: 4 in, 6 out]
          n53 = Array Subset(array=w126, index (col)=4 ("index"), length (col)=16 ("length")) -> (w123:u32[][])  [unwired: 2 in]
          n54 = call <vilib>:"Flatten Pixmap.vi"("24-bit pixmap"=w123) -> ("image data"=w121:T8)  [unwired: 10 in]
        }
        n55 = Bundle By Name(cluster=w99, "InterfaceSelection"=w104, "InterfaceIcons"=w109, "InterfaceInfo"=w96) -> (w113:T7)
        n56 = Build Array (concatenate)(T8 {"image type"=0, "image depth"=0, "image"=[], "mask"=[], "colors"=[], "Rectangle"={"left"=0, "top"=0, "right"=0, "bottom"=0}} ("image data"), w102, w112) -> (w106:T8[])
        n57 = invoke on="InterfaceList" class="MCListbox (strict)" method="Custom Item Symbols.Set Symbol Array"(error in=w111, "symbols"=w106) -> (error out=w107:errorcluster)  [unwired: 2 in, 3 out]
      }
      frame "UpdateSelection" {
        # "Change some selection to Grey if: The any child interface is selected (Blue)"
        n58 = Unbundle By Name(w152) -> ("InterfaceSelection"=w150:enum16{"Empty", "Not", "Grey", "Blue"}[], "InterfaceInfo"=w149:T3[])
        n59 = for {
          tunnel: w149 -> [w157] mode=indexing
          tunnel: [w156] -> w148 mode=indexing
          tunnel: [w154] -> w147 mode=indexing
          n60 = Unbundle By Name(w157) -> ("FullQualifierName"=w156:string, "ParentInterfaceFullQualifierNames"=w155:string[])
          n61 = Bundle("ParentInterfaceFullQualifierNames"=w155) -> (w154:T13)  [unwired: 1 in]
        }
        n62 = for {
          tunnel: w150 -> [w163] mode=indexing
          shift-right: [w158] -> w146
          shift-left: w150 -> [w159]
          tunnel: w149 -> [w162] mode=indexing
          tunnel: w148 -> [w161]
          tunnel: w147 -> [w160]
          n63 = case shown="\"Blue\"" w163 {
            tunnel: w162 -> [_ w171]
            tunnel: w161 -> [_ w170]
            tunnel: w160 -> [_ w168]
            tunnel: w159 -> [w164 w167]
            tunnel: [w164 w165] -> w158
            frame Default {
            }
            frame "Blue" {
              # "Change all parent interfaces to Grey"
              n64 = Unbundle By Name(w171) -> ("ParentInterfaceFullQualifierNames"=w169:string[])
              n65 = while {
                tunnel: w170 -> [w181]
                shift-right: [w177] -> _
                shift-left: w169 -> [w180]
                tunnel: w168 -> [w178]
                tunnel: [w176] -> w166 mode=concatenating
                stop <- w179 stop-if-true
                n66 = for {
                  tunnel: w181 -> [w187]
                  tunnel: w180 -> [w186] mode=indexing
                  tunnel: [w184] -> w176 mode=indexing
                  tunnel: w178 -> [w185]
                  tunnel: [w182] -> w177 mode=concatenating
                  n67 = Search 1D Array(1D array=w187, element=w186) -> (index of element=w184:i32)  [unwired: 1 in]
                  n68 = Index Array(array=w185, index=w184) -> (element=w183:T13)
                  n69 = Unbundle(w183) -> ("ParentInterfaceFullQualifierNames"=w182:string[])
                }
                n70 = Empty Array?(array=w177) -> (empty?=w179:bool)
              }
              n71 = for {
                shift-right: [w174] -> w165
                shift-left: w167 -> [w175]
                tunnel: w166 -> [w173] mode=indexing
                n72 = Replace Array Subset(array=w175, new element=enum16{"Empty", "Not", "Grey", "Blue"}."Grey", index=w173) -> (w174:enum16{"Empty", "Not", "Grey", "Blue"}[])
              }
            }
          }
        }
        n73 = Bundle By Name(cluster=w152, "InterfaceSelection"=w146) -> (w151:T7)
        n74 = call <resource>:"GDSString_AddStatesToQueue.vi"("State(s) in Front (\"\")"="ChangeGreyToBlue?" ("State(s) in Front (\"\")"), "State(s) in (\"\")"=w145) -> ("States Out"=w144:string)  [unwired: 13 in]
      }
      frame "UpdateInterfaceList" {
        n75 = Unbundle By Name(w193) -> ("InterfaceIcons"=w217:path[], "InterfaceInfo"=w218:T3[])
        n76 = Unbundle By Name(w193) -> ("Path"=w191:path)
        n77 = local read "InterfaceFilter"() -> (w209:string)
        n78 = call <vilib>:"Trim Whitespace.vi"("string"=w209) -> ("trimmed string"=w213:string)  [unwired: 1 in]
        n79 = To Lower Case(string=w213) -> (all lower case string=w212:string)
        n80 = Empty String/Path?(string/path=w213) -> (empty?=w216:bool)
        n81 = Equal?(x=w213, y="Interface name filter" ("InterfaceFilter")) -> (x = y?=w215:bool)
        n82 = Compound Arithmetic op=OR(w216, w215) -> (w214:bool)
        n83 = for {
          tunnel: [w248] -> w197 mode=indexing if=w235
          tunnel: w218 -> [w238] mode=indexing
          tunnel: w217 -> [w246]
          tunnel: [w245] -> w204 mode=indexing if=w235
          tunnel: w214 -> [w244]
          tunnel: w212 -> [w242]
          tunnel: [w237] -> w189 mode=indexing if=w235
          tunnel: [w236] -> w192 mode=indexing if=w235
          i -> [w237]
          n84 = Unbundle By Name(w238) -> ("IconPath"=w247:path, "Name(Short if no Conflicts)"=w243:string, "Description"=w230:string, "ParentInterfaceNames(Short if no Conflitcs)"=w240:string[])
          n85 = Unbundle By Name(w238) -> ("Path"=w236:path)
          n86 = call "GDSString_RemoveExtension.vim"("NameWithExtension"=w240) -> ("NameWithoutExtension"=w239:string[])  [unwired: 9 in, 1 out]
          n87 = case shown="False" w244 {
            tunnel: [w254 TRUE] -> w235
            tunnel: w243 -> [w257 _]
            tunnel: w242 -> [w256 _]
            frame False {
              n88 = To Lower Case(string=w257) -> (all lower case string=w253:string)
              n89 = Match Pattern(string=w253, regular expression=w256) -> (offset past match=w255:i32)  [unwired: 1 in, 3 out]
              n90 = Greater Or Equal To 0?(x=w255) -> (x >= 0?=w254:bool)
            }
            frame True {
            }
          }
          n91 = Array To Spreadsheet String(delimiter (Tab)=",", array=w239, 3:"%s" ("format string")) -> (spreadsheet string=w250:string)
          n92 = call <vilib>:"Trim Whitespace.vi"("string"=w250) -> ("trimmed string"=w249:string)  [unwired: 1 in]
          n93 = call <vilib>:"Trim Whitespace.vi"("string"=w230) -> ("trimmed string"=w234:string)  [unwired: 1 in]
          n94 = call <vilib>:"Search and Replace Pattern.vi"("string"=w234, "regular expression (\"\")"="[\\n\\r]+" ("regular expression (\"\")"), "replace string (\"\")"=" " ("replace string (\"\")"), "replace all? (F)"=TRUE) -> ("result string"=w229:string)  [unwired: 1 in, 1 out]
          n95 = Search 1D Array(1D array=w246, element=w247) -> (index of element=w245:i32)  [unwired: 1 in]
          n96 = Build Array("" ("element"), w243, w249, w229) -> (w248:string[])
        }
        n97 = Unbundle By Name(w193) -> ("InterfaceSelection"=w200:enum16{"Empty", "Not", "Grey", "Blue"}[])
        n98 = Search 1D Array(1D array=w192, element=w191) -> (index of element=w190:i32)  [unwired: 1 in]
        n99 = case shown="-1" w190 {
          selector: w190 -> [w222 _]
          tunnel: [w221 _] -> w188
          frame 0, Default {
            n100 = Build Array(w222) -> (w221:i32[])
          }
          frame -1 {
          }
        }
        n101 = Bundle By Name(cluster=w193, "VisiableInterfaceIndexes"=w189, "DisabledInterafaces"=w188) -> (w203:T7)
        n102 = call "Is Value Changed.vim"("value"=w197) -> ("changed or first call?"=w194:bool)
        n103 = property on="InterfaceList" class="MCListbox (strict)"("ItemNames"=w197, "Value"=i32[] [] ("_SelectInterfaceClass"), "DisabledItems"=w188) -> (error out=w196:errorcluster)  [unwired: 2 in, 1 out]
        n104 = case shown="True" w194 {
          tunnel: [w223 w224] -> w195
          tunnel: w196 -> [w223 w224]
          frame False {
          }
          frame True {
            n105 = property on="InterfaceList" class="MCListbox (strict)"("TopLeft"=T10 {"Row"=0, "Column"=0} ("Top Left Visible Cell")) -> ()  [unwired: 2 in, 2 out]
          }
        }
        n106 = Add(x=w204, y=4) -> (x+y=w205:i32[])
        n107 = for {
          tunnel: w189 -> [w227] mode=indexing
          tunnel: w200 -> [w228]
          tunnel: [w226] -> w198 mode=indexing
          n108 = Index Array(array=w228, index=w227) -> (element=w226:enum16{"Empty", "Not", "Grey", "Blue"})
        }
        n109 = property on="InterfaceList" class="MCListbox (strict)"(error in=w195, "ActiveCell"=T9 {"Row"=-2, "Column"=0} ("Active Cell:Active Cell"), "Symbols Vis"=TRUE ("Visible Items:Symbols Visible"), "ItemSyms"=w205) -> (error out=w199:errorcluster)  [unwired: 1 in, 1 out]
        n110 = property on="InterfaceList" class="MCListbox (strict)"(error in=w199, "ActiveCell"=T9 {"Row"=-2, "Column"=1} ("Active Cell:Active Cell"), "Symbols Vis"=TRUE ("Visible Items:Symbols Visible"), "ItemSyms"=w198) -> ()  [unwired: 1 in, 2 out]
      }
      frame "Update" {
        n111 = Unbundle By Name(w263) -> ("InterfaceSelection"=w281:enum16{"Empty", "Not", "Grey", "Blue"}[], "InterfaceInfo"=w293:T3[])
        n112 = Unbundle By Name(w263) -> ("StartInterfaceSelection"=w279:bool[], "ParentInterfaces(path)"=w284:path[], "Interfaces(MethodsImplemented)"=w285:cluster{"Methods":string[]}[])
        n113 = Unbundle By Name(w263) -> ("InterfacesParentClasesUses(path)"=w262:path[])
        n114 = Equal?(x=w281, y=enum16{"Empty", "Not", "Grey", "Blue"}."Blue") -> (x = y?=w278:bool[])
        n115 = for {
          tunnel: w293 -> [w335] mode=indexing
          tunnel: w281 -> [w336] mode=indexing
          tunnel: [w335] -> w265 mode=indexing if=w331
          tunnel: [w334] -> w283 mode=indexing
          tunnel: [w333] -> w282 mode=indexing
          tunnel: [w332] -> w264 mode=indexing if=w331
          i -> [w332]
          n116 = Unbundle By Name(w335) -> ("FullQualifierName"=w333:string, "Path"=w334:path)
          n117 = case shown="\"Grey\", \"Blue\"" w336 {
            tunnel: [_ TRUE] -> w331
            frame Default {
            }
            frame "Grey", "Blue" {
            }
          }
        }
        n118 = for {
          tunnel: w285 -> [w330] mode=indexing
          tunnel: w284 -> [w329] mode=indexing
          tunnel: w283 -> [w328]
          tunnel: w282 -> [w326]
          tunnel: [w323] -> w269 mode=indexing
          n119 = Unbundle By Name(w330) -> ("Methods"=w324:string[])
          n120 = Search 1D Array(1D array=w328, element=w329) -> (index of element=w327:i32)  [unwired: 1 in]
          n121 = Index Array(array=w326, index=w327) -> (element=w325:string)
          n122 = Bundle("FullQualifierName"=w325, "Methods"=w324) -> (w323:T14)  [unwired: 1 in]
        }
        n123 = Unbundle By Name(w263) -> ("IsInterface?"=w270:bool)
        n124 = Array Size(array=w262) -> (size(s)=w261:i32)
        n125 = Select(t=w269, s=w270, f=T11 [] ("StartSelectedMethodsPerInterfaces")) -> (s? t:f=w268:T11)
        n126 = control-ref of="Tree"() -> (w292:refnum<vi>)
        n127 = call <resource>:"CreateMethodTree.vi"("DisabledMethodsNames"=w269, "error in (no error)"=w290, "StartSelectedMethodsPerInterfaces"=w268, "InterfacePath"=w265, "TreeControlRef"=w292) -> ("error out"=w291:errorcluster, "InterfacesTag"=w286:string[], "MethodsTagPerInterfaces"=w287:cluster{"Array":string[]}[], "MethodsSelectedPerInterface"=w288:cluster{"Array":bool[]}[], "MethodsDisabledPerInterface"=w266:cluster{"Array":bool[]}[])  [unwired: 2 in]
        n128 = for {
          tunnel: w279 -> [w320] mode=indexing
          tunnel: w278 -> [w321] mode=indexing
          tunnel: [w322] -> w277 mode=indexing
          tunnel: [w319] -> w272 mode=indexing
          n129 = Compound Arithmetic op=AND(w321, invert w320) -> (w319:bool)
          n130 = Compound Arithmetic op=AND(invert w321, w320) -> (w322:bool)
        }
        n131 = Boolean To (0,1)(Boolean=w277) -> (0, 1=w276:i16[])
        n132 = Boolean To (0,1)(Boolean=w272) -> (0, 1=w273:i16[])
        n133 = Add Array Elements(numeric array=w276) -> (sum=w275:i16)
        n134 = Add Array Elements(numeric array=w273) -> (sum=w274:i16)
        n135 = Bundle By Name(cluster=w263, "SelectedInterfaceIndex"=w264, "MethodsSelectedPerInt"=w288, "MethodsPerInterfaces"=w287, "Interfaces"=w286, "MethodsDisabledPerInt"=w266) -> (w289:T7)
        n136 = case shown="1.." w274 {
          selector: w274 -> [_ w317]
          tunnel: [_ w316] -> w271
          frame 0, Default {
          }
          frame 1.. {
            n137 = Format Into String(format string="%d Added", w317) -> (resulting string=w316:string)  [unwired: 2 in, 1 out]
          }
        }
        n138 = case shown="1.." w275 {
          selector: w275 -> [_ w315]
          tunnel: [w307 w313] -> w260
          tunnel: w271 -> [w307 w310]
          frame 0, Default {
          }
          frame 1.. {
            n139 = Empty String/Path?(string/path=w310) -> (empty?=w312:bool)
            n140 = Concatenate Strings(w310, ", " ("string")) -> (w308:string)
            n141 = Select(t=w310, s=w312, f=w308) -> (s? t:f=w311:string)
            n142 = Format Into String(format string="%d Removed", initial string=w311, w315) -> (resulting string=w313:string)  [unwired: 1 in, 1 out]
          }
        }
        n143 = case shown="1.." w261 {
          selector: w261 -> [_ w297]
          tunnel: w260 -> [w295 w300]
          tunnel: [w295 w298] -> w259
          frame 0, Default {
          }
          frame 1.. {
            n144 = case shown="2.., Default" w297 {
              tunnel: ["are" ("string") "is" ("string")] -> w296
              frame 2.., Default {
              }
              frame 1 {
              }
            }
            n145 = Empty String/Path?(string/path=w300) -> (empty?=w301:bool)
            n146 = Concatenate Strings(w300, ", " ("string")) -> (w303:string)
            n147 = Select(t=w300, s=w301, f=w303) -> (s? t:f=w299:string)
            n148 = Format Into String(format string="%d %s Inherited", initial string=w299, w297, w296) -> (resulting string=w298:string)  [unwired: 1 in, 1 out]
          }
        }
        n149 = property on="InterfaceList" class="MCListbox (strict)"("Caption.Text"=w259) -> ()  [unwired: 2 in, 2 out]
      }
      frame "", "Idle" {
        n150 = event shown="[1] \"Cancel\", \"Save\": Value Change" {
          selector: _ -> [_ _ _ _ _ _ _]
          dyn-events: _ -> [_ _ _ _ _ _ _]
          timeout: _ -> [_ _ _ _ _ _ _]
          tunnel: ["Exit" "Exit" w361 _ "UpdateInterfaceList\nUpdate" _ _] -> w349
          tunnel: w345 -> [w350 w356 w362 w391 w395 w396 w398]
          tunnel: [w350 w355 w363 w387 w395 w396 w398] -> w348
          event Panel Close? {
            n151 = event-data() -> ()  [unwired: 1 in, 4 out]
            n152 = event-data("Discard?"=TRUE) -> ()  [unwired: 1 in, 1 out]
          }
          event "Cancel", "Save": Value Change {
            n153 = event-data() -> ()  [unwired: 1 in, 6 out]
            n154 = Bundle By Name(cluster=w356, "Cancel"="Cancel") -> (w355:T7)
          }
          event "InterfaceList": Mouse Down {
            n155 = event-data() -> ("Coords"=w373:T15)  [unwired: 1 in]
            n156 = Unbundle By Name(w362) -> ("DisabledInterafaces"=w359:i32[], "InterfaceSelection"=w365:enum16{"Empty", "Not", "Grey", "Blue"}[], "VisiableInterfaceIndexes"=w371:i32[])
            n157 = invoke on="InterfaceList" class="MCListbox (strict)" method="Point To Row Column"("Point"=w373) -> ("CellPosition"=w372:T9, "InGlyph"=w367:bool)  [unwired: 6 in, 5 out]
            n158 = Unbundle By Name(w372) -> ("Row"=w360:i32)
            n159 = Index Array(array=w371, index=w360) -> (element=w364:i32)
            n160 = Search 1D Array(1D array=w359, element=w360) -> (index of element=w358:i32)  [unwired: 1 in]
            n161 = Index Array(array=w365, index=w364) -> (element=w370:enum16{"Empty", "Not", "Grey", "Blue"})
            n162 = Less Than 0?(x=w358) -> (x < 0?=w357:bool)
            n163 = Not Equal?(x=w370, y=enum16{"Empty", "Not", "Grey", "Blue"}."Grey") -> (x != y?=w368:bool)
            n164 = Compound Arithmetic op=AND(w368, w367, w357) -> (w366:bool)
            n165 = case shown="False" w366 {
              tunnel: w365 -> [_ w380]
              tunnel: w364 -> [_ w379]
              tunnel: w362 -> [w374 w378]
              tunnel: [w374 w376] -> w363
              tunnel: [_ "UpdateSelection\nUpdateInterfaceList\nUpdate"] -> w361
              frame False {
              }
              frame True {
                n166 = in-place {
                  w383 = enum16{"Empty", "Not", "Grey", "Blue"}."Blue" ("y")
                  n167 = in-place-array #1(w380, w379) -> (w385:enum16{"Empty", "Not", "Grey", "Blue"})
                  n168 = Equal?(x=w385, y=w383) -> (x = y?=w384:bool)
                  n169 = Select(t=enum16{"Empty", "Not", "Grey", "Blue"}."Not" ("y"), s=w384, f=w383) -> (s? t:f=w381:enum16{"Empty", "Not", "Grey", "Blue"})
                  n170 = in-place-array #1(w381) -> (w377:enum16{"Empty", "Not", "Grey", "Blue"}[])  [unwired: 1 out]
                }
                n171 = Bundle By Name(cluster=w378, "InterfaceSelection"=w377) -> (w376:T7)
              }
            }
          }
          event "Tree": Mouse Down {
            n172 = event-data() -> ("CtlRef"=w392:refnum<vi>, "Coords"=w393:T15)  [unwired: 1 in]
            n173 = Unbundle By Name(w391) -> ("MethodsSelectedPerInt"=w390:cluster{"Array":bool[]}[], "MethodsPerInterfaces"=w389:cluster{"Array":string[]}[], "Interfaces"=w388:string[])
            n174 = call <resource>:"ChangeMethodTreeSelection.vi"("TreeControl in"=w392, "Interfaces"=w388, "MethodsPerInterfaces"=w389, "MouseClickCoordinates"=w393, "SelectedMethodsIn"=w390) -> ("SelectedMethodsOut"=w386:cluster{"Array":bool[]}[])  [unwired: 6 in]
            n175 = Bundle By Name(cluster=w391, "MethodsSelectedPerInt"=w386) -> (w387:T7)
          }
          event "InterfaceFilter": Value Change {
            n176 = event-data() -> ()  [unwired: 1 in, 6 out]
          }
          event "Help": Value Change {
            n177 = event-data() -> ()  [unwired: 1 in, 6 out]
            n178 = call <resource>:"GOOP_HelpMain.vi"() -> ()  [unwired: 12 in]
          }
          event "_ShowContextHelp": Value Change {
            n179 = event-data() -> ("NewVal"=w397:bool)  [unwired: 1 in]
            n180 = Control Help Window(1:w397) -> ()  [unwired: 1 in]
          }
        }
        n181 = Unbundle By Name(w345) -> ("MethodsSelectedPerInt"=w344:cluster{"Array":bool[]}[], "MethodsDisabledPerInt"=w343:cluster{"Array":bool[]}[])
        n182 = control-ref of="Tree"() -> (w346:refnum<vi>)
        n183 = call <resource>:"SetMethodTreeCaption.vi"("MethodsDisabledPerInt"=w343, "MethodsSelectedPerInt"=w344, "TreeControl in"=w346) -> ("Methods will be created"=w342:bool)  [unwired: 8 in]
        n184 = Select(t="Save and create methods", s=w342, f="Save changes") -> (s? t:f=w341:string)
        n185 = Build Array(w341) -> (w340:string[])
        n186 = property on="Save" class="Bool"("Strings [4]"=w340) -> ()  [unwired: 2 in, 2 out]
      }
      frame "ChangeGreyToBlue?" {
        (unwired) enum16{"Empty", "Not", "Grey", "Blue"}."Grey"
        # "If grey and no child of this is selected, change to Blue"
        n187 = Unbundle By Name(w413) -> ("InterfacesParentClasesUses(path)"=w399:path[], "InterfaceSelection"=w404:enum16{"Empty", "Not", "Grey", "Blue"}[], "InterfaceInfo"=w408:T3[])
        n188 = for {
          tunnel: w408 -> [w418] mode=indexing
          tunnel: [w417] -> w407 mode=indexing
          tunnel: [w415] -> w406 mode=indexing
          n189 = Unbundle By Name(w418) -> ("FullQualifierName"=w417:string, "ParentInterfaceFullQualifierNames"=w416:string[])
          n190 = Bundle("ParentInterfaceFullQualifierNames"=w416) -> (w415:T13)  [unwired: 1 in]
        }
        n191 = for {
          tunnel: w408 -> [w427] mode=indexing
          tunnel: [w419] -> w411 mode=concatenating if=w424
          tunnel: w404 -> [w426] mode=indexing
          tunnel: w407 -> [w423]
          tunnel: w406 -> [w422]
          n192 = Unbundle By Name(w427) -> ("ParentInterfaceFullQualifierNames"=w420:string[])
          n193 = Equal?(x=w426, y=enum16{"Empty", "Not", "Grey", "Blue"}."Blue") -> (x = y?=w424:bool)
          n194 = case shown="True" w424 {
            tunnel: w420 -> [_ w431]
            tunnel: w423 -> [_ w430]
            tunnel: w422 -> [_ w429]
            tunnel: [_ w428] -> w421
            frame False {
            }
            frame True {
              n195 = while {
                shift-right: [w432] -> _
                shift-left: w431 -> [w437]
                tunnel: [w435] -> _
                tunnel: w430 -> [w434]
                tunnel: w429 -> [w433]
                tunnel: [w432] -> w428 mode=concatenating
                stop <- w436 stop-if-true
                n196 = for {
                  tunnel: w437 -> [w443] mode=indexing
                  tunnel: [w442] -> w435 mode=indexing
                  tunnel: [w438] -> w432 mode=concatenating
                  tunnel: w434 -> [w441]
                  tunnel: w433 -> [w440]
                  n197 = Search 1D Array(1D array=w441, element=w443) -> (index of element=w442:i32)  [unwired: 1 in]
                  n198 = Index Array(array=w440, index=w442) -> (element=w439:T13)
                  n199 = Unbundle(w439) -> ("ParentInterfaceFullQualifierNames"=w438:string[])
                }
                n200 = Empty Array?(array=w432) -> (empty?=w436:bool)
              }
            }
          }
          n201 = Build Array (concatenate)(w420, w421) -> (w419:string[])
        }
        n202 = for {
          tunnel: w404 -> [w448] mode=indexing
          tunnel: w408 -> [w447] mode=indexing
          tunnel: w411 -> [w446]
          tunnel: [w445] -> w405 mode=indexing
          tunnel: w399 -> [w444]
          n203 = case shown="\"Grey\"" w448 {
            selector: w448 -> [w449 _]
            tunnel: w447 -> [_ w459]
            tunnel: w446 -> [_ w458]
            tunnel: [w449 w462] -> w445
            tunnel: w444 -> [_ w455]
            frame Default {
            }
            frame "Grey" {
              # "Should we change this to Blue?"
              n204 = Unbundle By Name(w459) -> ("Path"=w454:path, "FullQualifierName"=w457:string)
              n205 = Search 1D Array(1D array=w455, element=w454) -> (index of element=w453:i32)  [unwired: 1 in]
              n206 = Greater Or Equal To 0?(x=w453) -> (x >= 0?=w452:bool)
              n207 = Search 1D Array(1D array=w458, element=w457) -> (index of element=w456:i32)  [unwired: 1 in]
              n208 = Greater Or Equal To 0?(x=w456) -> (x >= 0?=w451:bool)
              n209 = Or(x=w452, y=w451) -> (x .or. y?=w450:bool)
              n210 = Select(t=enum16{"Empty", "Not", "Grey", "Blue"}."Grey", s=w450, f=enum16{"Empty", "Not", "Grey", "Blue"}."Blue") -> (s? t:f=w462:enum16{"Empty", "Not", "Grey", "Blue"})
            }
          }
        }
        n211 = Not Equal?(x=w404, y=w405) -> (x != y?=w403:bool)
        n212 = Select(t="UpdateSelection" ("State(s) in Front (\"\")"), s=w403, f="") -> (s? t:f=w401:string)
        n213 = Bundle By Name(cluster=w413, "InterfaceSelection"=w405) -> (w412:T7)
        n214 = call <resource>:"GDSString_AddStatesToQueue.vi"("State(s) in Front (\"\")"=w401, "State(s) in (\"\")"=w410) -> ("States Out"=w409:string)  [unwired: 13 in]
      }
      frame "Error", "Exit", Default {
        # "Change INterfaceToImplent Type Def\n1) Add/RemoveList\n2) Add/RemoveMethodList"
        # "Add all interfaces that was not in the StartInterfaceSelectionList (or in the Inherited list)\nRemove all interfaces that is not in the StartSelectionList"
        n215 = Unbundle By Name(w471) -> ("MethodsSelectedPerInt"=w465:cluster{"Array":bool[]}[], "MethodsDisabledPerInt"=w473:cluster{"Array":bool[]}[], "SelectedInterfaceIndex"=w472:i32[])
        n216 = Unbundle By Name(w471) -> ("InterfaceInfo"=w474:T3[], "InterfaceSelection"=w463:enum16{"Empty", "Not", "Grey", "Blue"}[])
        n217 = Unbundle By Name(w471) -> ("StartInterfaceSelection"=w477:bool[])
        n218 = Unbundle By Name(w471) -> ("LvClasses"=w470:refnum<vi>[], "LvInterfaces"=w469:refnum<vi>[])
        n219 = Build Array (concatenate)(w470, w469) -> (w468:refnum<vi>[])
        n220 = for {
          tunnel: w477 -> [w485] mode=indexing
          tunnel: w474 -> [w507] mode=indexing
          tunnel: [w493] -> w476 mode=indexing if=w482
          tunnel: [w493] -> w475 mode=indexing if=w506
          tunnel: w473 -> [w502]
          tunnel: [w503] -> w464 mode=indexing if=w484
          tunnel: w472 -> [w500]
          tunnel: w465 -> [w498]
          tunnel: w463 -> [w486] mode=indexing
          i -> [w499]
          n221 = Search 1D Array(1D array=w500, element=w499) -> (index of element=w497:i32)  [unwired: 1 in]
          n222 = Index Array(array=w498, index=w497) -> (element=w496:cluster{"Array":bool[]})
          n223 = Index Array(array=w502, index=w497) -> (element=w501:cluster{"Array":bool[]})
          n224 = Unbundle(w496) -> ("Array"=w495:bool[])
          n225 = Unbundle(w501) -> ("Array"=w504:bool[])
          n226 = Unbundle By Name(w507) -> ("Methods"=w505:T4[], "Path"=w493:path)
          n227 = Equal?(x=w486, y=enum16{"Empty", "Not", "Grey", "Blue"}."Grey") -> (x = y?=w488:bool)
          n228 = for {
            tunnel: w505 -> [w512] mode=indexing
            tunnel: w504 -> [w509] mode=indexing
            tunnel: [w511] -> w492 mode=indexing if=w508
            tunnel: w495 -> [w510] mode=indexing
            n229 = Compound Arithmetic op=AND(w510, invert w509) -> (w508:bool)
            n230 = Unbundle By Name(w512) -> ("Name"=w511:string)
          }
          n231 = Equal?(x=w486, y=enum16{"Empty", "Not", "Grey", "Blue"}."Blue") -> (x = y?=w483:bool)
          n232 = Compound Arithmetic op=OR(w488, w483) -> (w487:bool)
          n233 = Compound Arithmetic op=AND(w483, invert w485) -> (w482:bool)
          n234 = Compound Arithmetic op=AND(invert w483, w485) -> (w506:bool)
          n235 = Bundle(cluster=T12 {"InterfacePath"=path "", "Methods"=[]} ("Methods"), "InterfacePath"=w493, "Methods"=w492) -> (w503:T12)
          n236 = Empty Array?(array=w492) -> (empty?=w491:bool)
          n237 = Compound Arithmetic op=AND(invert w491, w487) -> (w484:bool)
        }
        n238 = Close Reference(reference=w468) -> ()  [unwired: 1 in, 1 out]
        n239 = Bundle By Name(cluster=T1 {"InterfaceToAdd(Path)"=[], "InterfaceToRemove(Path)"=[], "MethodsToAddPerInterface(Empty=>All)"=[], "MethodsToRemovePerInterface(Empty=>All)"=[]} ("HanldeInterfacesData"), "MethodsToAddPerInterface(Empty=>All)"=w464, "InterfaceToAdd(Path)"=w476, "InterfaceToRemove(Path)"=w475) -> (w466:T1)
        n240 = Bundle By Name(cluster=w471, "HandleInterfacesData"=w466) -> (w478:T7)
      }
    }
  }
  "error out" <- w21
  n241 = Generate User Event(user event=w11, event data cluster="Stop" ("Stop")) -> (user event out=w16:refnum<user-event>)  [unwired: 2 in, 1 out]
  n242 = Destroy User Event(user event=w16) -> ()  [unwired: 1 in, 1 out]
  n243 = Unbundle By Name(w8) -> ("Cancel"=→"Cancelled":bool, "HandleInterfacesData"=→"HanldeInterfacesData":T1)
  n244 = call <resource>:"GDSString_AddStatesToQueue.vi"() -> ()  [unwired: 15 in, 1 out]
  "ClassWriterNativeOut" <- "ClassWriterNativeIn"
